vi "Biot-Savart_3_axis.vi"() -> ()   [LabVIEW 2024]
panel:
  out "OK?":bool
  out "phi":dbl(knob) scale=0.0..360.0
  out "theta":dbl(knob) scale=0.0..180.0
  in  "Bbgz":dbl
  in  "Bbgy":dbl
  in  "Bbgx":dbl
  in  "sz":dbl=0.2286
  in  "sy":dbl=0.1651
  in  "sx":dbl=0.1905
  in  "az":dbl=0.4191
  in  "ay":dbl=0.3048
  in  "ax":dbl=0.39116
  in  "Nz":dbl=20.0
  in  "Ny":dbl=10.0
  in  "Nx":dbl=15.0
  in  "phi_deg":dbl
  in  "theta_deg":dbl
  in  "Bmg_mT":dbl
  in  "Imax":dbl
  out "kz":dbl
  out "ky":dbl
  out "kx":dbl
  out "Iz":dbl
  out "Iy":dbl
  out "Ix":dbl
  out "Waveform Graph":dbl[](graph)
  out "output variable":dbl[](array[numeric])
  # "in m"
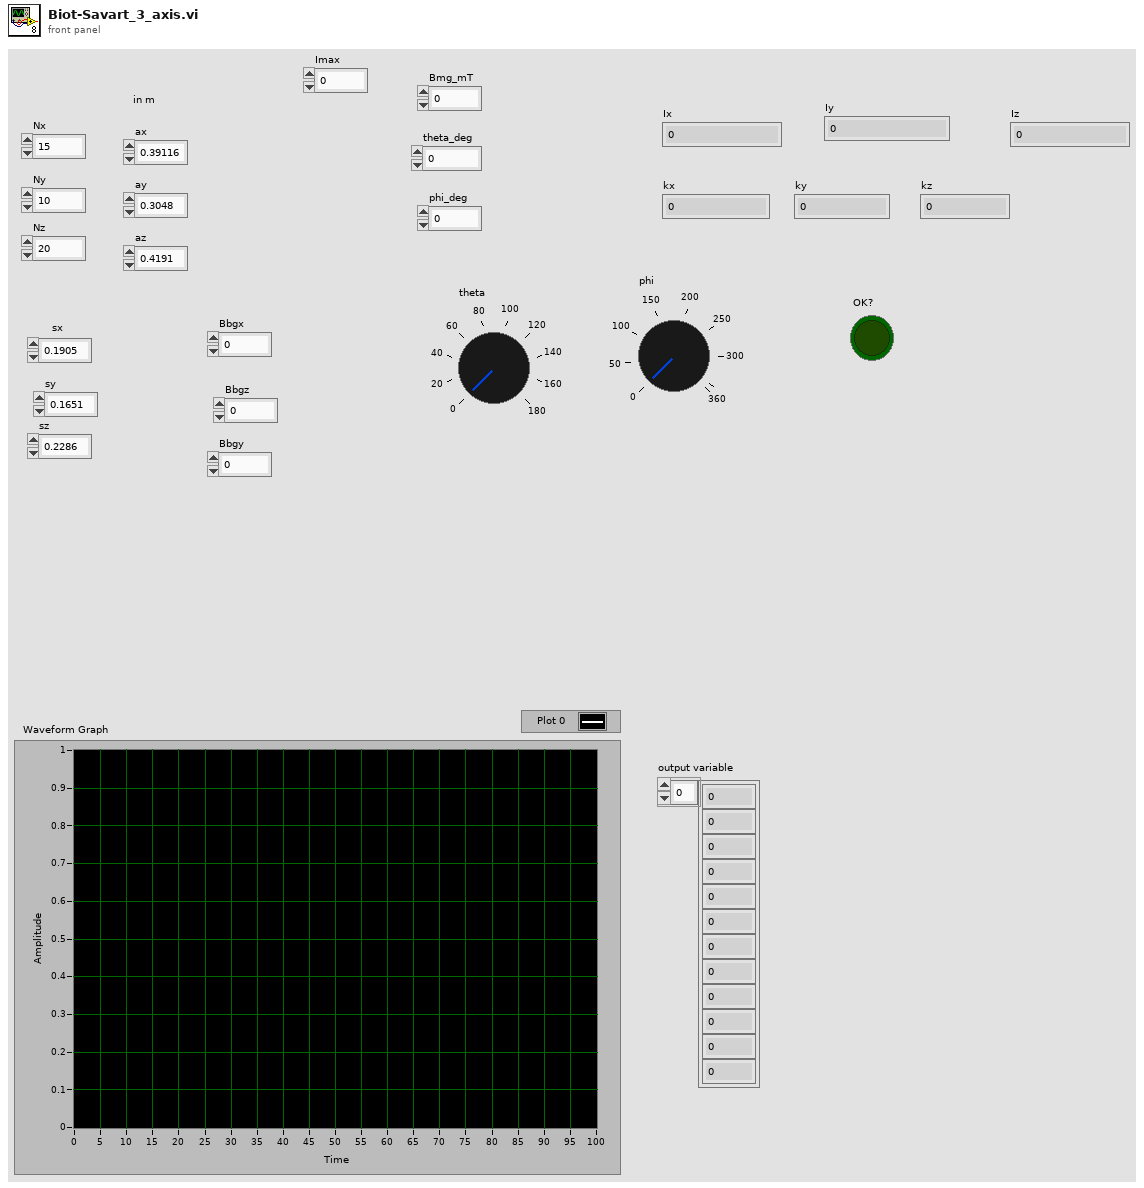
[diagram p1: front panel]
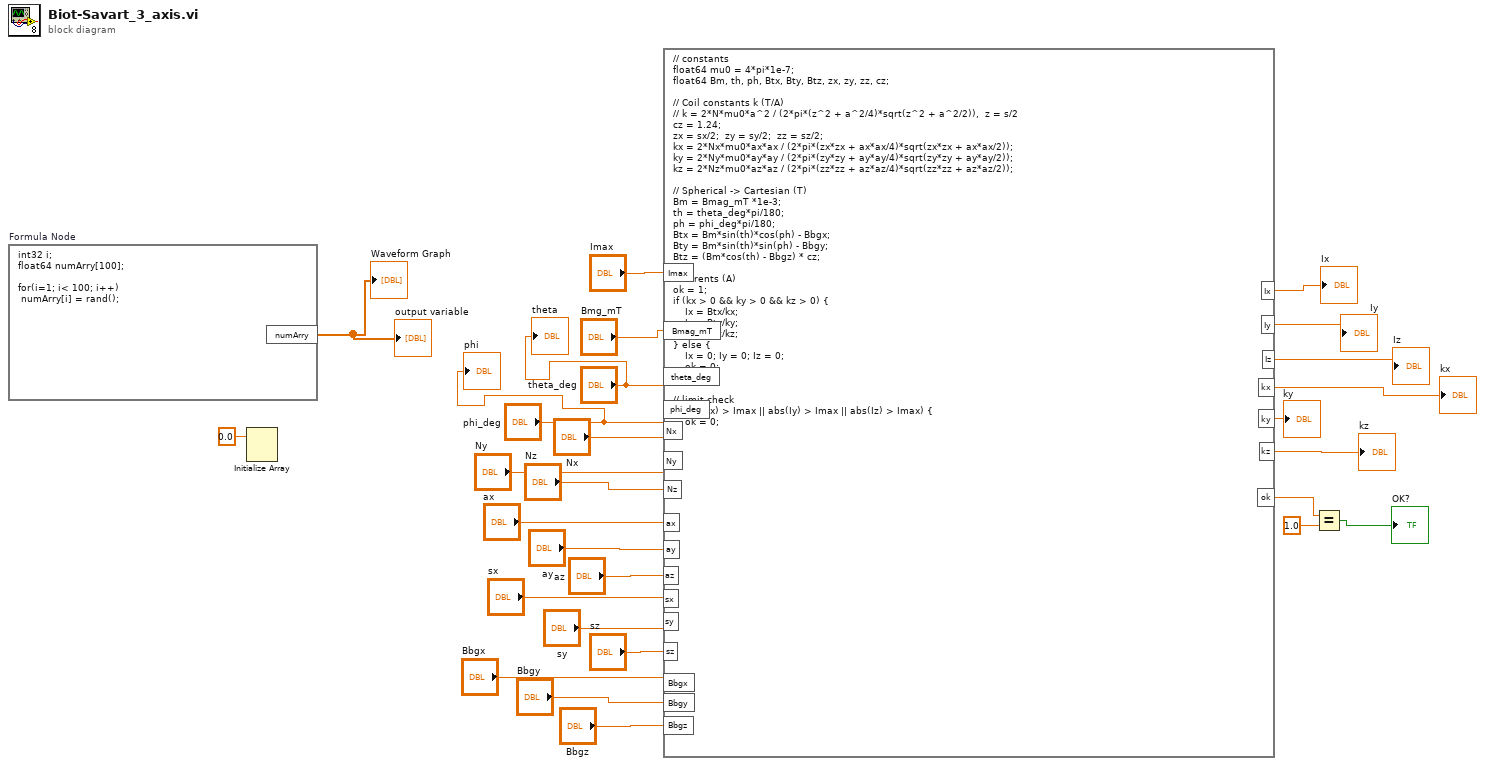
[diagram p0: block diagram]
diagram:
  n1 = formula code="int32 i;\nfloat64 numArry[100];\n\nfor(i=1; i< 100; i++)\n numArry[i] = rand();"() -> ("numArry"=→"output variable" →"Waveform Graph":dbl[])
  n2 = Initialize Array "Initialize Array"(0.0 ("element")) -> ()  [unwired: 2 in, 1 out]
  n3 = formula code="// constants\nfloat64 mu0 = 4*pi*1e-7; \nfloat64 Bm, th, ph, Btx, Bty, Btz, zx, zy, zz, cz;\n\n// Coil constants k (T/A)\n// k = 2*N*mu0*a^2 / (2*pi*(z^2 + a^2/4)*sqrt(z^2 + a^2/2)),  z = s/2\ncz = 1.24;\nzx = sx/2;  zy = sy/2;  zz = sz/2;\nkx = 2*Nx*mu0*ax*ax / (2*pi*(zx*zx + ax*ax/4)*sqrt(zx*zx + ax*ax/2));\nky = 2*Ny*mu0*ay*ay / (2*pi*(zy*zy + ay*ay/4)*sqrt(zy*zy + ay*ay/2));\nkz = 2*Nz*mu0*az*az / (2*pi*(zz*zz + az*az/4)*sqrt(zz*zz + az*az/2));\n\n// Spherical -> Cartesian (T)\nBm = Bmag_mT *1e-3;\nth = theta_deg*pi/180;\nph = phi_deg*pi/180;\nBtx = Bm*sin(th)*cos(ph) - Bbgx;\nBty = Bm*sin(th)*sin(ph) - Bbgy;\nBtz = (Bm*cos(th) - Bbgz) * cz;\n\n//currents (A)\nok = 1;\nif (kx > 0 && ky > 0 && kz > 0) {\n    Ix = Btx/kx;\n    Iy = Bty/ky;\n    Iz = Btz/kz;\n} else {\n    Ix = 0; Iy = 0; Iz = 0;\n    ok = 0;       \n}\n\n// limit check\nif (abs(Ix) > Imax || abs(Iy) > Imax || abs(Iz) > Imax) {\n    ok = 0;\n}"("theta_deg"="theta_deg", "phi_deg"="phi_deg", "Nx"="Nx", "Ny"="Ny", "Nz"="Nz", "ax"="ax", "ay"="ay", "az"="az", "sx"="sx", "sy"="sy", "sz"="sz", "Bbgx"="Bbgx", "Bbgy"="Bbgy", "Bbgz"="Bbgz", "Imax"="Imax", "Bmag_mT"="Bmg_mT") -> ("Ix"=→"Ix":dbl, "Iy"=→"Iy":dbl, "Iz"=→"Iz":dbl, "kx"=→"kx":dbl, "ky"=→"ky":dbl, "kz"=→"kz":dbl, "ok"=w3:dbl)
  n4 = Equal?(x=w3, y=1.0) -> (x = y?=→"OK?":bool)
  "theta" <- "theta_deg"
  "phi" <- "phi_deg"
